vi "Scan Engine RemIO Module Page.vi"(8 "error in (no error)":errorcluster, 11 "Node Ptr":T1 format="%.0x") -> (0 "error out":errorcluster)   [LabVIEW 2020, in "SEECD System Explorer.lvlib"]
uses:
  SEECD System Explorer.lvlib
  <vilib>/NI VeriStand/Custom Device API/Custom Device Item Ref.ctl
  Includes/Modules.lvlibp/RSI Module/SubPanel Command.ctl
  Includes/Modules.lvlibp/RemIO Module/RemIO Module.lvclass
  <vilib>/NI VeriStand/Custom Device API/Custom Device API.lvlib
  Includes/Modules.lvlibp/RSI Module/RSI Module.lvclass
panel:
  out "Module Name":string
  out "Module Index":u8
  in  "Header":cluster{"Section Name":string}={"Section Name"="Module Settings"}
  in  "Description":string
  out "Name":string
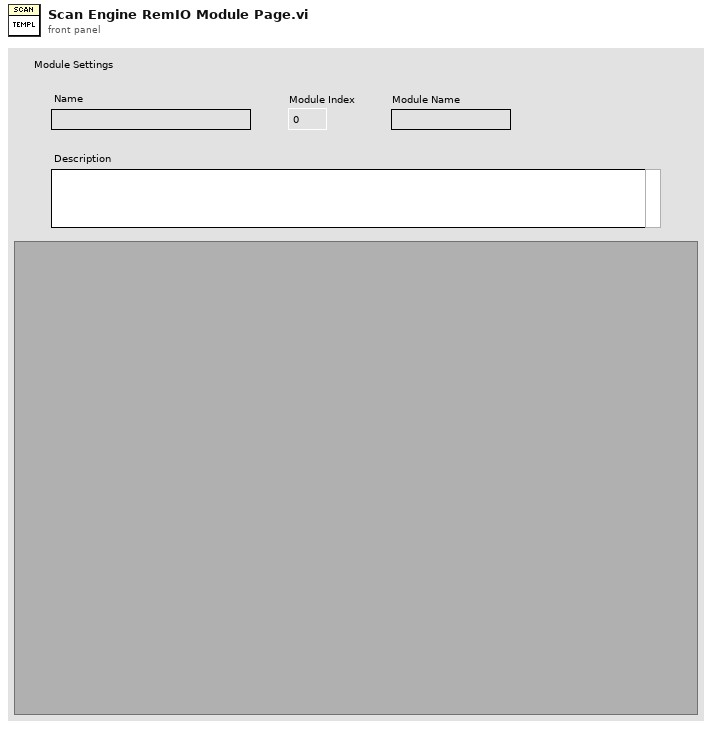
[diagram p1: front panel]
types:
  T1 = typedef "Custom Device API.lvlib/Custom Device Item Ref.ctl" = u64
  T2 = typedef "Custom Device API.lvlib/Custom Device Item Info.ctl" = cluster{"Name":string, "Is Channel":bool, "GUID":string, "Is Waveform":bool}
  T3 = typedef "Modules.lvlibp/Custom Device API.lvlib/Custom Device Item Ref.ctl" = u64
  T4 = typedef "Modules.lvlibp/RSI Module.lvclass/SubPanel Command.ctl" = enum16{"Stop"}
  T5 = typedef "Custom Device API.lvlib/Custom Device Commands.ctl" = enum16{"Default", "Item renamed", "Shutdown", "Dynamic button pressed"}
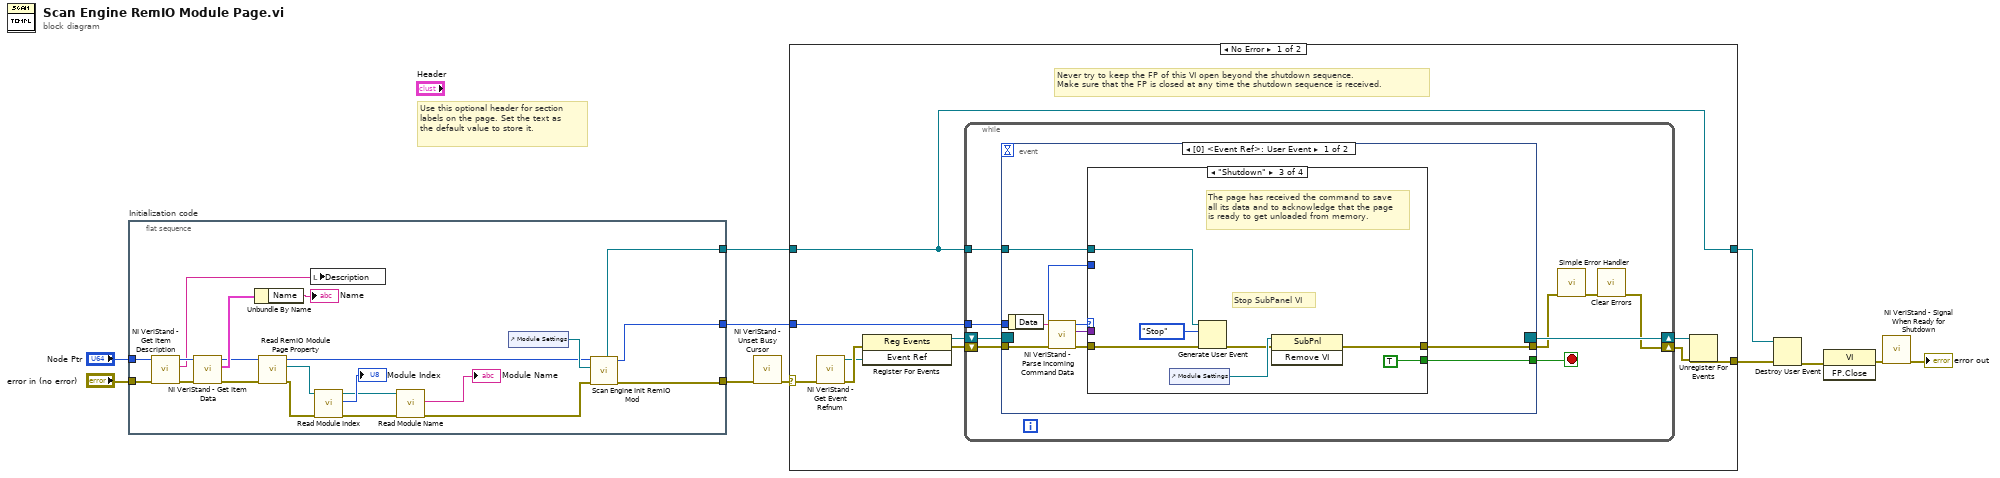
[diagram p0: block diagram]
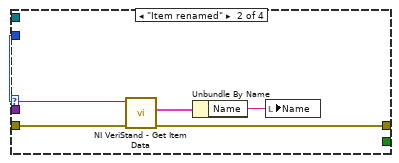
[diagram p3: hidden frame]
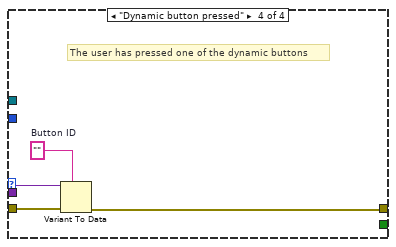
[diagram p4: hidden frame]
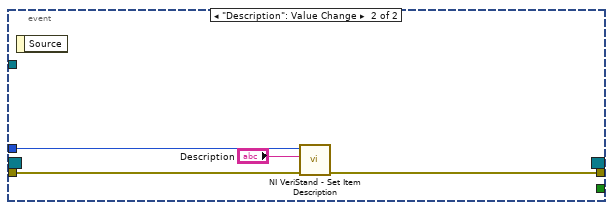
[diagram p5: hidden frame]
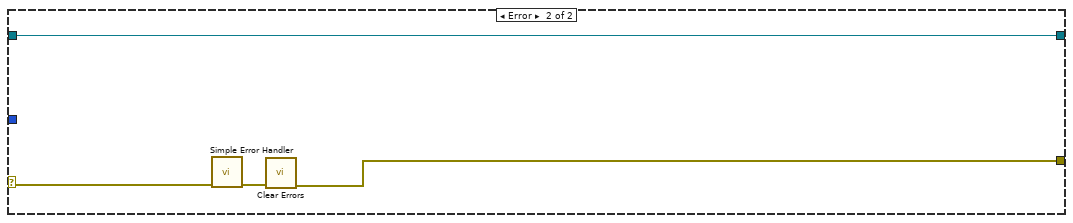
[diagram p6: hidden frame]
diagram:
  # "Use this optional header for section labels on the page. Set the text as the default value to store it."
  n1 = flat-sequence "Initialization code" {
    tunnel: "error in (no error)" -> [w26]
    tunnel: "Node Ptr" -> [w27]
    tunnel: [w22] -> w8
    tunnel: [w25] -> w5
    tunnel: [w23] -> w4
    frame #0 {
      n2 = call <vilib>:"NI VeriStand - Get Item Description.vi"("error in (no error)"=w26, "Item Ref in"=w27) -> ("error out"=w30:errorcluster, "Description"=w31:string, "Item Ref out"=w32:T1)  [unwired: 7 out]
      n3 = call <vilib>:"NI VeriStand - Get Item Data.vi"("error in (no error)"=w30, "Item Ref in"=w32) -> ("error out"=w20:errorcluster, "Item Info"=w29:T2, "Item Ref out"=w21:T1)  [unwired: 7 out]
      n4 = Unbundle By Name(w29) -> ("Name"=→"Name":string)
      n5 = call "Read RemIO Module Page Property.vi"("error in (no error)"=w20, "Node Ptr In"=w21) -> ("error out"=w17:errorcluster, "RemIO Module"=w18:refnum<class "RemIO Module.lvclass">, "Node Ptr Out"=w19:T3)  [unwired: 7 in]
      n6 = local write "Description"(w31) -> ()
      n7 = call-dynamic "Read Module Index.vi"("error in (no error)"=w17, "RemIO Module in"=w18) -> ("error out"=w15:errorcluster, "Module Index"=→"Module Index":u8, "RemIO Module out"=w13:refnum<class "RemIO Module.lvclass">)  [unwired: 7 in]
      n8 = call-dynamic "Read Module Name.vi"("error in (no error)"=w15, "RemIO Module in"=w13) -> ("error out"=w14:errorcluster, "Module Name"=→"Module Name":string)  [unwired: 7 in, 1 out]
      n9 = control-ref of="Module Settings"() -> (w24:refnum<vi>)
      n10 = call "Scan Engine Init RemIO Mod.vi"("error in (no error)"=w14, "SubPanel Ref"=w24, "Node Ptr In"=w19) -> ("error out"=w22:errorcluster, "Node Ptr Out"=w25:T1, "SubPanel Command"=w23:refnum<user-event>)  [unwired: 6 in]
    }
  }
  n11 = call <vilib>:"NI VeriStand - Unset Busy Cursor.vi"("error in (no error)"=w8) -> ("error out"=w7:errorcluster)  [unwired: 10 out]
  n12 = case shown="No Error" w7 {
    selector: w7 -> [w34 w85]
    tunnel: [w39 w83] -> w2
    tunnel: w5 -> [w35 _]
    tunnel: w4 -> [w33 w82]
    tunnel: [w33 w82] -> w3
    frame No Error {
      # "Never try to keep the FP of this VI open beyond the shutdown sequence.\nMake sure that the FP is closed at any time the shutdown sequence is received."
      n13 = call <vilib>:"NI VeriStand - Get Event Refnum.vi"("error in (no error)"=w34) -> ("error out"=w42:errorcluster, "Event Ref"=w38:refnum<user-event>)  [unwired: 9 out]
      n14 = register-events(error in=w42, w38) -> (reference out=w36:refnum<event-registration>, error out=w37:errorcluster)  [unwired: 1 in]
      n15 = while {
        tunnel: w35 -> [w47]
        shift-right: [w44] -> w40
        shift-left: w37 -> [w50]
        shift-right: [w51] -> w41
        shift-left: w36 -> [w49]
        tunnel: w33 -> [w43]
        stop <- w48 stop-if-true
        n16 = event shown="[0] <Event Ref>: User Event" {
          selector: w49 -> [_ _]
          dyn-events: [_ _] -> w51
          timeout: _ -> [_ _]
          tunnel: w50 -> [w60 w80]
          tunnel: [w56 _] -> w48
          tunnel: [w55 w79] -> w46
          tunnel: w47 -> [w54 w81]
          tunnel: w43 -> [w52 _]
          event User Event {
            n17 = event-data() -> ("Data"=w59:string)  [unwired: 1 out]
            n18 = call <vilib>:"NI VeriStand - Parse Incoming Command Data.vi"("error in (no error)"=w60, "Incoming data"=w59) -> ("error out"=w58:errorcluster, "Outgoing data"=w53:variant, "Action"=w57:T5)  [unwired: 7 out]
            n19 = case shown="\"Shutdown\"" w57 {
              tunnel: w58 -> [w61 w66 w70 w77]
              tunnel: [_ _ TRUE _] -> w56
              tunnel: [w61 w63 w67 w74] -> w55
              tunnel: w54 -> [_ w65 _ _]
              tunnel: w53 -> [_ _ _ w76]
              tunnel: w52 -> [_ _ w72 _]
              frame "Default", Default {
              }
              frame "Item renamed" {
                n20 = call <vilib>:"NI VeriStand - Get Item Data.vi"("error in (no error)"=w66, "Item Ref in"=w65) -> ("error out"=w63:errorcluster, "Item Info"=w64:T2)  [unwired: 8 out]
                n21 = Unbundle By Name(w64) -> ("Name"=w62:string)
                n22 = local write "Name"(w62) -> ()
              }
              frame "Shutdown" {
                # "Stop SubPanel VI"
                # "The page has received the command to save all its data and to acknowledge that the page is ready to get unloaded from memory."
                n23 = control-ref of="Module Settings"() -> (w69:refnum<vi>)
                n24 = Generate User Event(user event=w72, event data cluster=SubPanel_Command."Stop" ("event data"), error in=w70) -> (error out=w68:errorcluster)  [unwired: 1 in, 1 out]
                n25 = invoke class="SubPnl" method="Remove VI"(reference=w69, error in=w68) -> (error out=w67:errorcluster)  [unwired: 1 in, 2 out]
              }
              frame "Dynamic button pressed" {
                w75 = ""  # Button ID
                # "The user has pressed one of the dynamic buttons"
                n26 = Variant To Data(error in=w77, type=w75, Variant=w76) -> (error out=w74:errorcluster)  [unwired: 1 out]
              }
            }
          }
          event "Description": Value Change {
            n27 = event-data() -> ()  [unwired: 2 out]
            n28 = call <vilib>:"NI VeriStand - Set Item Description.vi"("error in (no error)"=w80, "Description"="Description", "Item Ref in"=w81) -> ("error out"=w79:errorcluster)  [unwired: 8 out]
          }
        }
        n29 = call <vilib>:"Simple Error Handler.vi"("error in (no error)"=w46) -> ("error out"=w45:errorcluster)  [unwired: 1 in, 7 out]
        n30 = call <vilib>:"Clear Errors.vi"("error in (no error)"=w45) -> ("error out"=w44:errorcluster)  [unwired: 1 in, 5 out]
      }
      n31 = Unregister For Events(event registration refnum=w41, error in=w40) -> (error out=w39:errorcluster)
    }
    frame Error {
      n32 = call <vilib>:"Simple Error Handler.vi"("error in (no error)"=w85) -> ("error out"=w84:errorcluster)  [unwired: 1 in, 7 out]
      n33 = call <vilib>:"Clear Errors.vi"("error in (no error)"=w84) -> ("error out"=w83:errorcluster)  [unwired: 1 in, 5 out]
    }
  }
  n34 = Destroy User Event(user event=w3, error in=w2) -> (error out=w1:errorcluster)
  n35 = invoke class="VI" method="FP.Close"(error in=w1) -> (error out=w11:errorcluster)  [unwired: 2 in, 2 out]
  n36 = call <vilib>:"NI VeriStand - Signal When Ready for Shutdown.vi"("error in (no error)"=w11) -> ("error out"=→"error out":errorcluster)  [unwired: 10 out]
